vi "Read Job Report Event.vi"(8 "error in (no error)":errorcluster, 11 "Job in":refnum<class "Job.lvclass">) -> (0 "error out":errorcluster, 1 "Job Started Event":refnum<user-event>, 2 "Job Report Event":refnum<user-event>, 3 "Job out":refnum<class "Job.lvclass">, 4 "Job Update Event":refnum<user-event>)   [LabVIEW 2013, in "openCronJob.lvlib" / "Job.lvclass"]
uses:
  Job.lvclass
  JobReport/JobReport.lvclass
  Job Started -- cluster.ctl
  Job Update -- cluster.ctl
  Job.lvclass/Job.ctl
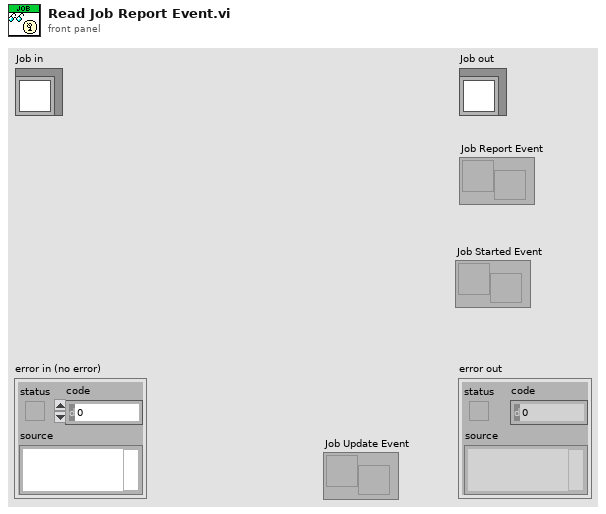
[diagram p1: front panel]
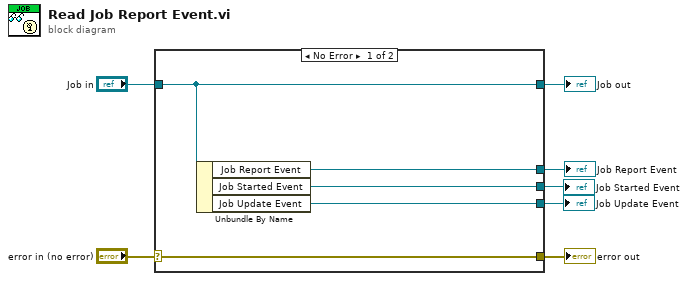
[diagram p0: block diagram]
diagram:
  n1 = case shown="No Error" "error in (no error)" {
    selector: "error in (no error)" -> [w12 w13]
    tunnel: [w12 w13] -> w6
    tunnel: [w11 w14] -> w4
    tunnel: "Job in" -> [w11 w14]
    tunnel: [w10 _] -> w3
    tunnel: [w9 _] -> w2
    tunnel: [w8 _] -> w1
    frame No Error {
      n2 = Unbundle By Name(w11) -> ("Job Report Event"=w10:refnum<user-event>, "Job Started Event"=w9:refnum<user-event>, "Job Update Event"=w8:refnum<user-event>)
    }
    frame Error {
    }
  }
  "error out" <- w6
  "Job out" <- w4
  "Job Report Event" <- w3
  "Job Started Event" <- w2
  "Job Update Event" <- w1
